vi "Measurement Logic.vi"() -> ()   [LabVIEW 2022 SP3, in "Single Tone - Digital Mic.lvlib"]
uses:
  Single Tone - Digital Mic.lvlib
  <vilib>/Plug-In SDKs/Measurements/Measure Call Context/Measure Call Context.lvclass
  Measurement Configuration.ctl
  shared/measurements/controls/lowpass filter.ctl
  shared/measurements/controls/weighting filter.ctl
  shared/measurements/controls/highpass filter.ctl
  shared/measurements/controls/measurement units.ctl
  Measurement Results.ctl
  <vilib>/addons/_NISVFA/_Generation/Signal Generation/SV Signal/sv_System Timing Model.ctl
  shared/Stop Variable Action.ctl
  <vilib>/PDM Acquisition Toolkit/host/Classes/Tasks/PDM Tasks/Controls/Acquisition Mode.ctl
  <vilib>/PDM Acquisition Toolkit/shared/controls/clock mode.ctl
  shared/measurements/controls/audio filter settings.ctl
  shared/measurements/controls/single tone microphone measurement settings.ctl
  shared/measurements/controls/units settings - mic.ctl
  <vilib>/DAQmx/read.llb/DAQmx Read (Analog Wfm 1Chan NSamp).vi
  <vilib>/DAQmx/write.llb/DAQmx Write (Analog Wfm 1Chan NSamp).vi
  <vilib>/addons/_NISVFA/_Generation/Signal Generation/SV Sinusoid/SV Sinusoid.lvclass
  C:/Program Files/National Instruments/LabVIEW 2022/vi.lib/addons/_NISVFA/_Generation/Signal Generation/SV Signal/SV Signal.lvclass
  <vilib>/addons/_NISVFA/_Generation/Signal Generation/SV Sinusoid/Configure Sine.vi
  <vilib>/DAQmx/create/channels.llb/DAQmx Create Channel (AO-Voltage-Basic).vi
  <vilib>/DAQmx/configure/timing.llb/DAQmx Timing (Sample Clock).vi
  <vilib>/DAQmx/configure/events/hardwareSignals.llb/DAQmx Export Signal (Most Signals).vi
  <vilib>/addons/_NISVFA/_Generation/Signal Generation/SV Signal/Write Sample Rate.vi
  <vilib>/addons/_NISVFA/_Generation/Signal Generation/SV Signal/Write System Timing Model.vi
  <vilib>/addons/_NISVFA/_Generation/Signal Generation/SV Signal/Write Ramp Parameters.vi
  <vilib>/DAQmx/create/channels.llb/DAQmx Create Channel (AI-Sound Pressure-Microphone).vi
  <vilib>/Waveform/WDTOps.llb/WDT Waveform Duration DBL.vi
  <vilib>/DAQmx/configure/trigger.llb/DAQmx Start Trigger (Digital Edge).vi
  <vilib>/DAQmx/miscellaneous.llb/DAQmx Fill In Error Info.vi
  <vilib>/Waveform/WDTOps.llb/WDT Get Waveform Subset DBL.vi
  <vilib>/addons/_NISVFA/_Generation/Signal Generation/SV Signal/SV Signal.lvclass
  <resource>/objmgr/daqmx.rc
  shared/combined digital api/Combo Digital Audio API.lvlib
  <vilib>/PDM Acquisition Toolkit/host/Classes/Tasks/PDM Tasks/PDM Task.lvclass
  <vilib>/PDM Acquisition Toolkit/shared/PDM Shared.lvlib
panel:
  out "calculated microphone sensitivity (dBFS)":dbl
  out "measurement results":T1={"channel name"="Empty", "frequency (Hz)"=0.0, "amplitude (Pa RMS)"=0.0, "amplitude (dBSPL)"=0.0, "microphone sensitivity (dBFS)"=0.0, "SNR"=0.0, "THD+N"=0.0, "THD"=0.0, "wfm - dt"=0.0, "wfm - data"=[0.0], "fft - f0"=0.0, "fft - df"=0.0, "fft - data"=[0.0], "ref mic wfm - dt"=0.0, "ref mic wfm - data"=[0.0]}
  in  "measurement configuration":T2={"digital channel list"="Lorem ipsum dolor sit", "input cfg file"="", "digital mic sensitivity (dBFS)"=1.2, "ref mic channel"="7821\\PCMo 0", "ref mic sensitivity (mV/Pa)"=32.0, "output channel"="7821\\PCMo 0", "signal frequency"=64.0, "output level (dBSPL)"=-32.0, "output voltage ratio"=-64.0, "lowpass filter"=enum."No filter", "weighting filter"=enum."A-weighting", "highpass filter"=enum."AC", "band start"=1.0, "band stop"=1.0, "min measurement cycles"=20, "min measurement time (s)"=0.1, "min settling cycles"=0, "min settling time (s)"=0.0, "SNR units"=enum."dB", "THD+N units"=enum."dB", "THD units"=enum."dB"} {"output voltage ratio" format="%#_g Pa/V"; "signal frequency" format="%#_13g"; "digital mic sensitivity (dBFS)" format="%#_13g"}
  out "measure call context out":refnum<class "Measure Call Context.lvclass">
  in  "measure call context in":refnum<class "Measure Call Context.lvclass">
  out "error out":errorcluster
  in  "error in":errorcluster
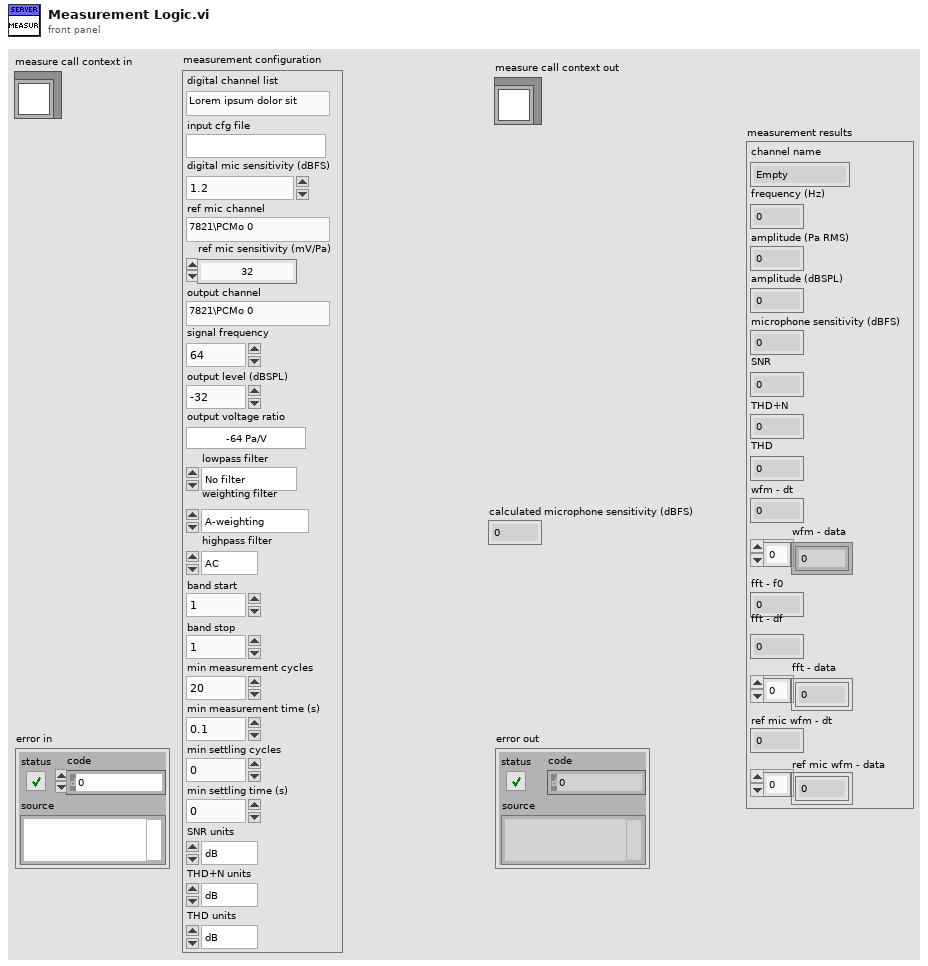
[diagram p1: front panel]
types:
  T1 = typedef "Single Tone - Digital Mic.lvlib/Measurement Results.ctl" = cluster{"channel name":string, "frequency (Hz)":dbl, "amplitude (Pa RMS)":dbl, "amplitude (dBSPL)":dbl, "microphone sensitivity (dBFS)":dbl, "SNR":dbl, "THD+N":dbl, "THD":dbl, "wfm - dt":dbl, "wfm - data":dbl[], "fft - f0":dbl, "fft - df":dbl, "fft - data":dbl[], "ref mic wfm - dt":dbl, "ref mic wfm - data":dbl[]}
  T2 = typedef "Single Tone - Digital Mic.lvlib/Measurement Configuration.ctl" = cluster{"digital channel list":string, "input cfg file":string, "digital mic sensitivity (dBFS)":dbl, "ref mic channel":string, "ref mic sensitivity (mV/Pa)":dbl, "output channel":string, "signal frequency":dbl, "output level (dBSPL)":dbl, "output voltage ratio":dbl, "lowpass filter":T3, "weighting filter":T4, "highpass filter":T5, "band start":dbl, "band stop":dbl, "min measurement cycles":u32, "min measurement time (s)":dbl, "min settling cycles":u32, "min settling time (s)":dbl, "SNR units":T6, "THD+N units":T6, "THD units":T6}
  T3 = typedef "lowpass filter.ctl" = enum32{"No filter", "AES17 20kHz", "AES17 40kHz"}
  T4 = typedef "weighting filter.ctl" = enum32{"Linear", "A-weighting", "B-weighting", "C-weighting"}
  T5 = typedef "highpass filter.ctl" = enum32{"DC", "AC"}
  T6 = typedef "measurement units.ctl" = enum32{"dB", "%", "x/y"}
  T7 = typedef "units settings - mic.ctl" = cluster{"SNR units":T6, "THD+N units":T6, "THD units":T6}
  T8 = typedef "single tone microphone measurement settings.ctl" = cluster{"Band start":dbl, "Band stop":dbl, "Frequency":dbl}
  T9 = typedef "audio filter settings.ctl" = cluster{"weighting filter":T4, "highpass filter":T5, "lowpass filter ":T3}
  T10 = typedef "PDM Shared.lvlib/clock mode.ctl" = enum16{"divided clock", "DDS"}
  T11 = typedef "PDM Acquisition Class Library.lvlib/PDM Task.lvclass/Acquisition Mode.ctl" = enum16{"Finite", "Continuous"}
  T12 = typedef "Stop Variable Action.ctl" = enum16{"Reset", "Check", "Stop"}
  T13 = typedef "SV Signal.lvclass/sv_System Timing Model.ctl" = i64
  T14 = cluster{"profile":enum16{"Linear", "Half cosine"}, "durations [s]":cluster{"ramp-up":dbl, "transition":dbl, "ramp-down":dbl}}
  T15 = typedef "Combo Digital Audio API.lvlib/task.ctl" = cluster{"task ref":u64, "audio type":T16, "sample rate":dbl}
  T16 = typedef "input type.ctl" = enum32{"Digital Serial", "PDM"}
  T17 = typedef "single tone microphone measurements.ctl" = cluster{"channel":string, "frequency (Hz)":dbl, "amplitude (Pa rms)":dbl, "amplitude (dBSPL)":dbl, "SNR":dbl, "THD+N":dbl, "THD":dbl, "phase (deg)":dbl}
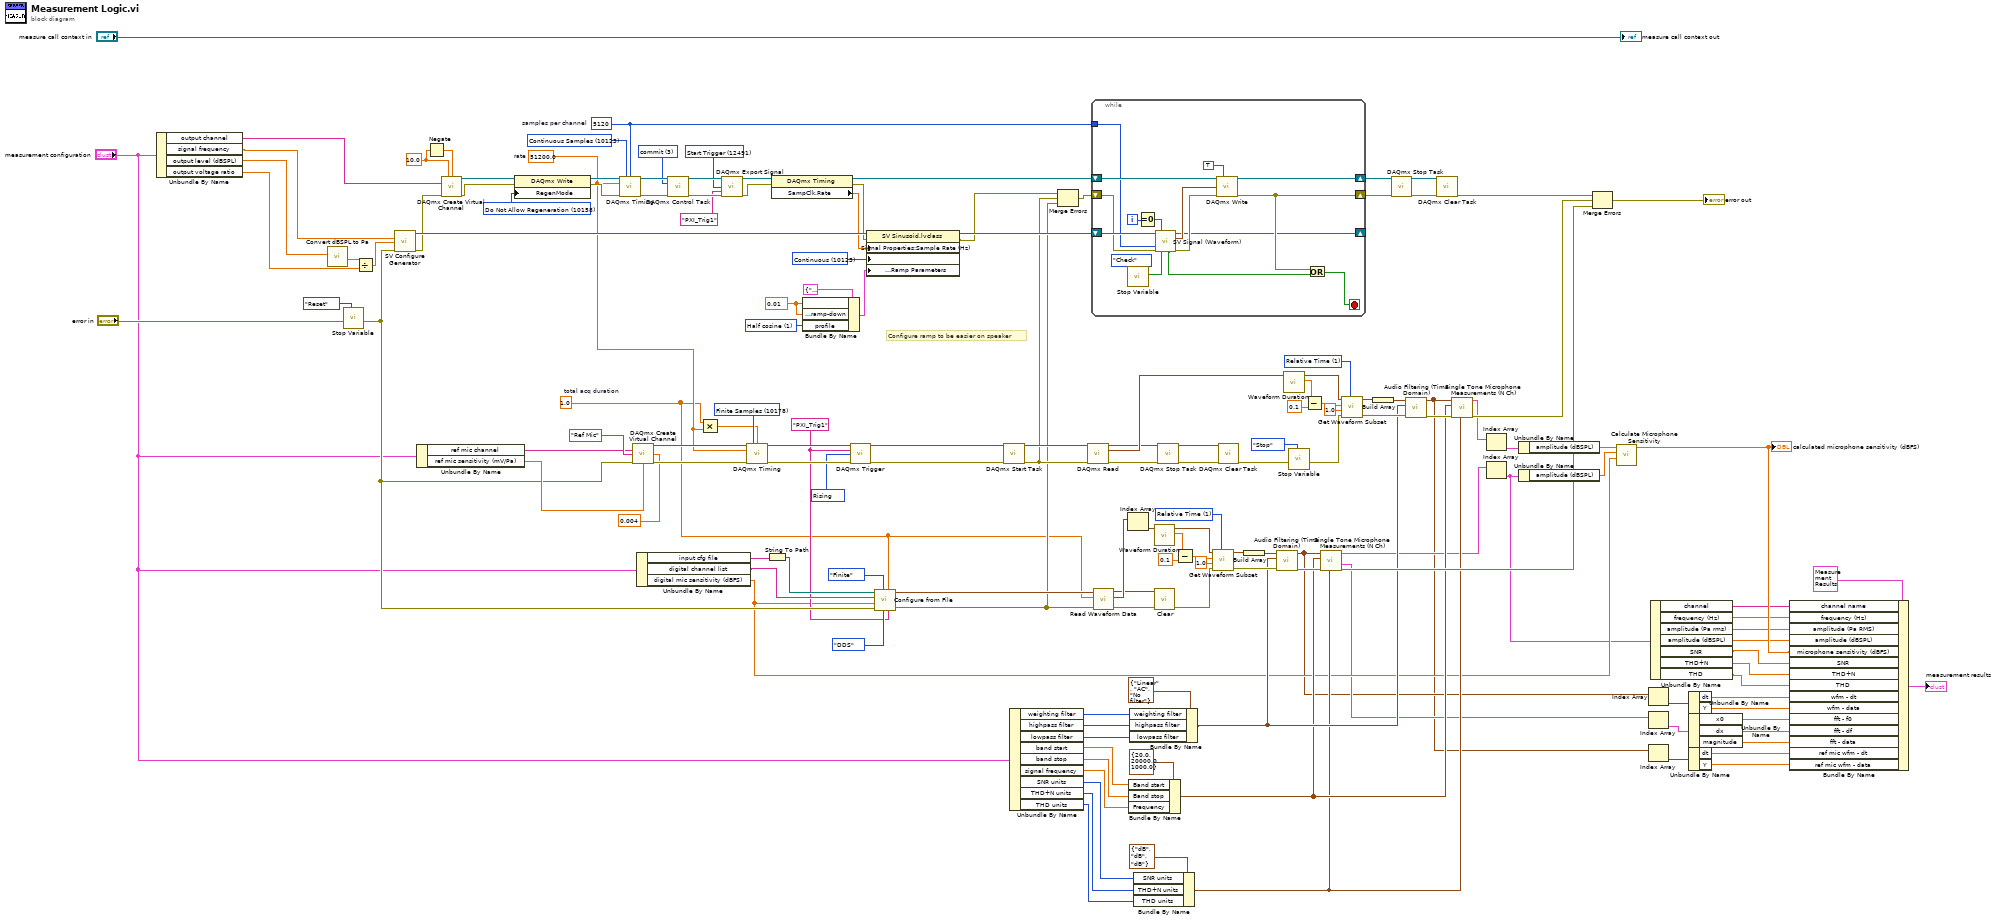
[diagram p0: block diagram]
diagram:
  w63 = u16 1 items=["Samples", "Relative Time"] ("start/duration format")
  w3 = 1.0  # total acq duration
  w92 = u16 1 items=["Samples", "Relative Time"] ("start/duration format")
  w104 = 10280 items=["Rising"=10280, "Falling"=10171] ("edge")
  w73 = "PXI_Trig1"
  w111 = 10178 items=["Finite Samples"=10178, "Continuous Samples"=10123] ("sample mode")
  w126 = 12491 items=["AI Convert Clock"=12484, "10MHz Reference Clock"=12536, "20MHz Timebase Clock"=12486, "Sample Clock"=12487, "Advance Trigger"=12488, "Reference Trigger"=12490, "Start Trigger"=12491, "Advance Complete Event"=12492, "AI Hold Complete Event"=12493, "Counter Output Event"=12494, "Change Detection Event"=12511, "Watchdog Timer Expired Event"=12512] ("signal")
  w131 = 3 items=["verify"=2, "reserve"=4, "commit"=3, "unreserve"=5, "abort"=6] ("action")
  w150 = 0.01 ("ramp duration")
  w148 = u16 1 items=["Linear", "Half cosine"] ("ramp profile")
  w142 = 10158 items=["Allow Regeneration"=10097, "Do Not Allow Regeneration"=10158] ("RegenMode")
  w145 = 10.0 ("maximum value")
  w112 = 5120  # samples per channel
  w146 = 10123 items=["Finite Samples"=10178, "Continuous Samples"=10123, "Hardware Timed Single Point"=12522] ("sample mode")
  w69 = 51200.0  # rate
  w147 = T13 10123 items=["Finite"=10178, "-"=-1, "Continuous"=10123, "-"=-2, "Settled"=110123, "Averaged"=210123, "Discrete Sweep"=310123, "Continuous Sweep"=410123] ("System Timing Model")
  # "Configure ramp to be easier on speaker"
  n1 = Unbundle By Name("measurement configuration") -> ("output channel"=w122:string, "signal frequency"=w121:dbl, "output level (dBSPL)"=w120:dbl, "output voltage ratio"=w119:dbl)
  n2 = call "Convert dBSPL to Pa.vi"("dB SPL"=w120) -> ("Pa pk"=w135:dbl)  [unwired: 9 in, 1 out]
  n3 = call "Stop Variable.vi"("action"=Stop_Variable_Action."Reset", "error in (no error)"="error in") -> ("error out"=w77:errorcluster)  [unwired: 8 in, 1 out]
  n4 = Divide(x=w135, y=w119) -> (x/y=w134:dbl)
  n5 = call-poly <vilib>:"SV Configure Generator.vi"("frequency (Hz)"=w121, "amplitude"=w134, "error in (no error)"=w77) -> ("signal configuration"=w152:refnum<class "SV Sinusoid.lvclass">, "error out"=w143:errorcluster)  [unwired: 11 in]
  n6 = Unbundle By Name("measurement configuration") -> ("ref mic channel"=w102:string, "ref mic sensitivity (mV/Pa)"=w101:dbl)
  n7 = Negate(x=w145) -> (-x=w144:dbl)
  n8 = call-poly <vilib>:"DAQmx Create Virtual Channel.vi"("maximum value"=w145, "minimum value"=w144, "physical channels"=w122, "error in"=w143) -> ("task out"=w141:refnum<k21>, "error out"=w139:errorcluster)  [unwired: 10 in]
  n9 = property class="DAQmx Write"(reference=w141, error in=w139, "RegenMode"=w142) -> (reference out=w140:refnum<k21>, error out=w138:errorcluster)
  n10 = call-poly <vilib>:"DAQmx Timing.vi"("task/channels in"=w140, "sample mode"=w146, "samples per channel"=w112, "rate"=w69, "error in"=w138) -> ("task out"=w133:refnum<k21>, "error out"=w132:errorcluster)  [unwired: 9 in]
  n11 = call-poly <vilib>:"DAQmx Create Virtual Channel.vi"("physical channels"=w102, "name to assign"="Ref Mic", "current excitation value"=0.004, "error in"=w77, "microphone sensitivity"=w101) -> ("task out"=w110:refnum<k21>, "error out"=w109:errorcluster)  [unwired: 9 in]
  n12 = Unbundle By Name("measurement configuration") -> ("input cfg file"=w79:string, "digital channel list"=w76:string, "digital mic sensitivity (dBFS)"=w29:dbl)
  n13 = call <vilib>:"DAQmx Control Task.vi"("task/channels in"=w133, "action"=w131, "error in"=w132) -> ("task out"=w130:refnum<k21>, "error out"=w129:errorcluster)  [unwired: 11 in]
  n14 = Multiply(x=w3, y=w69) -> (x*y=w70:dbl)
  n15 = call-poly <vilib>:"DAQmx Export Signal.vi"("task/channels in"=w130, "signal"=w126, "output terminal"="PXI_Trig1", "error in"=w129) -> ("task out"=w128:refnum<k21>, "error out"=w127:errorcluster)  [unwired: 10 in]
  n16 = call-poly <vilib>:"DAQmx Timing.vi"("task/channels in"=w110, "sample mode"=w111, "samples per channel"=w70, "rate"=w69, "error in"=w109) -> ("task out"=w108:refnum<k21>, "error out"=w106:errorcluster)  [unwired: 9 in]
  n17 = String To Path(string=w79) -> (path=w78:path)
  n18 = property class="DAQmx Timing"(reference=w128, error in=w127) -> (reference out=w114:refnum<k21>, error out=w136:errorcluster, "SampClk.Rate"=w137:dbl)
  n19 = Bundle By Name(cluster=T14 {"profile"=enum."Linear", "durations [s]"={"ramp-up"=0.0, "transition"=0.0, "ramp-down"=0.0}} ("Ramp Parameters:All Elements"), "durations [s].ramp-up"=w150, "durations [s].ramp-down"=w150, "profile"=w148) -> (w149:T14)
  n20 = call-poly <vilib>:"DAQmx Trigger.vi"("task/channels in"=w108, "source"=w73, "edge"=w104, "error in"=w106) -> ("task out"=w107:refnum<k21>, "error out"=w105:errorcluster)  [unwired: 10 in]
  n21 = property class="SV Sinusoid.lvclass"(reference=w152, error in=w136, "Signal Properties:Sample Rate (Hz)"=w137, "Signal Properties:System Timing Model"=w147, "Signal Properties:Ramps:Ramp Parameters"=w149) -> (reference out=w113:refnum<class "SV Sinusoid.lvclass">, error out=w98:errorcluster)
  n22 = call "Configure from File.vi"("digital trigger"=w73, "acq duration (s)"=w3, "clock mode"=clock_mode."DDS", "acquisition mode"=Acquisition_Mode."Finite", "error in (no error)"=w77, "microphone sensitivity (dBFS)"=w29, "channels"=w76, "file path"=w78) -> ("error out"=w71:errorcluster, "task"=w72:T15)  [unwired: 2 in]
  n23 = call <vilib>:"DAQmx Start Task.vi"("task/channels in"=w107, "error in"=w105) -> ("task out"=w90:refnum<k21>, "error out"=w89:errorcluster)  [unwired: 12 in]
  n24 = Unbundle By Name("measurement configuration") -> ("weighting filter"=w47:T4, "highpass filter"=w46:T5, "lowpass filter"=w45:T3, "band start"=w42:dbl, "band stop"=w41:dbl, "signal frequency"=w1:dbl, "SNR units"=w2:T6, "THD+N units"=w36:T6, "THD units"=w35:T6)
  n25 = Merge Errors(w98, w89, w71) -> (w99:errorcluster)
  n26 = call-poly <vilib>:"DAQmx Read.vi"("task/channels in"=w90, "error in"=w89) -> ("task out"=w84:refnum<k21>, "data"=w91:waveform(dbl), "error out"=w51:errorcluster)  [unwired: 11 in]
  n27 = while {
    tunnel: w112 -> [w167]
    shift-right: [w165] -> w118
    shift-left: w114 -> [w169]
    shift-right: [w166] -> w117
    shift-left: w99 -> [w161]
    shift-right: [w160] -> _
    shift-left: w113 -> [w168]
    i -> [w157]
    stop <- w159 stop-if-true
    n28 = call "Stop Variable.vi"("action"=Stop_Variable_Action."Check") -> ("stop"=w155:bool)  [unwired: 9 in, 1 out]
    n29 = Equal To 0?(x=w157) -> (x = 0?=w158:bool)
    n30 = call-dynamic "SV Signal (Waveform).vi"("signal configuration"=w168, "reset"=w158, "samples"=w167, "error in (no error)"=w161, "stop"=w155) -> ("signal configuration"=w160:refnum<class "SV Sinusoid.lvclass">, "output waveform"=w163:waveform(dbl), "done"=w156:bool, "error out"=w164:errorcluster)  [unwired: 5 in, 2 out]
    n31 = call-poly <vilib>:"DAQmx Write.vi"("task/channels in"=w169, "auto start"=TRUE, "data"=w163, "error in"=w164) -> ("task out"=w165:refnum<k21>, "error out"=w166:errorcluster)  [unwired: 9 in, 1 out]
    n32 = Or(x=w166, y=w156) -> (x .or. y?=w159:bool)
  }
  n33 = call "Read Waveform Data.vi"("error in (no error)"=w71, "acq duration (s)"=w3, "task"=w72) -> ("error out"=w55:errorcluster, "waveforms"=w60:waveform(dbl)[], "task"=w54:T15)  [unwired: 6 in]
  n34 = Index Array(array=w60) -> (element=w61:waveform(dbl))  [unwired: 1 in]
  n35 = Bundle By Name(cluster=T8 {"Band start"=20.0, "Band stop"=20000.0, "Frequency"=1000.0} ("measurement settings"), "Band start"=w42, "Band stop"=w41, "Frequency"=w1) -> (w39:T8)
  n36 = Bundle By Name(cluster=T9 {"weighting filter"=enum."Linear", "highpass filter"=enum."AC", "lowpass filter "=enum."No filter"} ("filter settings"), "weighting filter"=w47, "highpass filter"=w46, "lowpass filter"=w45) -> (w40:T9)
  n37 = Bundle By Name(cluster=T7 {"SNR units"=enum."dB", "THD+N units"=enum."dB", "THD units"=enum."dB"} ("units settings"), "SNR units"=w2, "THD+N units"=w36, "THD units"=w35) -> (w37:T7)
  n38 = call-poly <vilib>:"Waveform Duration.vi"("waveform in"=w61) -> ("duration"=w68:dbl, "waveform out"=w64:waveform(dbl))  [unwired: 8 in, 1 out]
  n39 = call "Clear.vi"("error in (no error)"=w55, "task"=w54) -> ("error out"=w53:errorcluster)  [unwired: 9 in]
  n40 = call <vilib>:"DAQmx Stop Task.vi"("task/channels in"=w84, "error in"=w51) -> ("task out"=w88:refnum<k21>, "error out"=w87:errorcluster)  [unwired: 12 in]
  n41 = Subtract(x=w68, y=0.1) -> (x-y=w65:dbl)
  n42 = call-poly <vilib>:"Get Waveform Subset.vi"("start/duration format"=w63, "error in (no error)"=w53, "duration"=1.0, "start samples/time"=w65, "waveform in"=w64) -> ("error out"=w57:errorcluster, "waveform out"=w62:waveform(dbl))  [unwired: 1 in, 2 out]
  n43 = call <vilib>:"DAQmx Clear Task.vi"("task in"=w88, "error in"=w87) -> ("error out"=w85:errorcluster)  [unwired: 13 in]
  n44 = Build Array(w62) -> (w24:waveform(dbl)[])
  n45 = call "Audio Filtering (Time Domain).vi"("waveforms"=w24, "filter settings"=w40, "error in"=w57) -> ("time domain"=w22:waveform(dbl)[], "error out"=w56:errorcluster)  [unwired: 6 in]
  n46 = call-poly <vilib>:"Waveform Duration.vi"("waveform in"=w91) -> ("duration"=w97:dbl, "waveform out"=w93:waveform(dbl))  [unwired: 8 in, 1 out]
  n47 = call "Stop Variable.vi"("action"=Stop_Variable_Action."Stop", "error in (no error)"=w85) -> ("error out"=w50:errorcluster)  [unwired: 8 in, 1 out]
  n48 = Subtract(x=w97, y=0.1) -> (x-y=w94:dbl)
  n49 = call "Single Tone Microphone Measurements (N Ch).vi"("units settings"=w37, "error in"=w56, "measurement settings"=w39, "waveforms"=w22) -> ("error out"=w52:errorcluster, "spectra"=w23:cluster{"x0":dbl, "dx":dbl, "magnitude":dbl[]}[], "measurements"=w31:T17[])  [unwired: 4 in, 1 out]
  n50 = call-poly <vilib>:"Get Waveform Subset.vi"("start/duration format"=w92, "error in (no error)"=w50, "duration"=1.0, "start samples/time"=w94, "waveform in"=w93) -> ("error out"=w59:errorcluster, "waveform out"=w80:waveform(dbl))  [unwired: 1 in, 2 out]
  n51 = Build Array(w80) -> (w81:waveform(dbl)[])
  n52 = call <vilib>:"DAQmx Stop Task.vi"("task/channels in"=w118, "error in"=w117) -> ("task out"=w116:refnum<k21>, "error out"=w115:errorcluster)  [unwired: 12 in]
  n53 = call "Audio Filtering (Time Domain).vi"("waveforms"=w81, "filter settings"=w40, "error in"=w59) -> ("time domain"=w15:waveform(dbl)[], "error out"=w58:errorcluster)  [unwired: 6 in]
  n54 = call <vilib>:"DAQmx Clear Task.vi"("task in"=w116, "error in"=w115) -> ("error out"=w83:errorcluster)  [unwired: 13 in]
  n55 = call "Single Tone Microphone Measurements (N Ch).vi"("units settings"=w37, "error in"=w58, "measurement settings"=w39, "waveforms"=w15) -> ("error out"=w49:errorcluster, "measurements"=w34:T17[])  [unwired: 4 in, 2 out]
  n56 = Index Array(array=w34) -> (element=w33:T17)  [unwired: 1 in]
  n57 = Index Array(array=w31) -> (element=w11:T17)  [unwired: 1 in]
  n58 = Unbundle By Name(w33) -> ("amplitude (dBSPL)"=w32:dbl)
  n59 = Unbundle By Name(w11) -> ("amplitude (dBSPL)"=w30:dbl)
  n60 = Merge Errors(w83, w49, w52) -> (→"error out":errorcluster)
  n61 = call "Calculate Microphone Sensitivity.vi"("microphone sensitivity (dBFS)"=w29, "measured sound level (dBSPL)"=w30, "reference sound level (dBSPL)"=w32) -> ("calculated microphone sensitivity (dBFS)"=w12:dbl)  [unwired: 8 in]
  "calculated microphone sensitivity (dBFS)" <- w12
  n62 = Index Array(array=w22) -> (element=w26:waveform(dbl))  [unwired: 1 in]
  n63 = Index Array(array=w23) -> (element=w25:cluster{"x0":dbl, "dx":dbl, "magnitude":dbl[]})  [unwired: 1 in]
  n64 = Index Array(array=w15) -> (element=w16:waveform(dbl))  [unwired: 1 in]
  n65 = Unbundle By Name(w11) -> ("channel"=w10:string, "frequency (Hz)"=w9:dbl, "amplitude (Pa rms)"=w8:dbl, "amplitude (dBSPL)"=w7:dbl, "SNR"=w6:dbl, "THD+N"=w5:dbl, "THD"=w4:dbl)
  n66 = Unbundle By Name(w26) -> ("dt"=w21:dbl, "Y"=w20:dbl[])
  n67 = Unbundle By Name(w25) -> ("x0"=w19:dbl, "dx"=w18:dbl, "magnitude"=w17:dbl[])
  n68 = Unbundle By Name(w16) -> ("dt"=w14:dbl, "Y"=w13:dbl[])
  n69 = Bundle By Name(cluster=T1 {"channel name"="Empty", "frequency (Hz)"=0.0, "amplitude (Pa RMS)"=0.0, "amplitude (dBSPL)"=0.0, "microphone sensitivity (dBFS)"=0.0, "SNR"=0.0, "THD+N"=0.0, "THD"=0.0, "wfm - dt"=0.0, "wfm - data"=[0.0], "fft - f0"=0.0, "fft - df"=0.0, "fft - data"=[0.0], "ref mic wfm - dt"=0.0, "ref mic wfm - data"=[0.0]} ("measurement results"), "channel name"=w10, "frequency (Hz)"=w9, "amplitude (Pa RMS)"=w8, "amplitude (dBSPL)"=w7, "microphone sensitivity (dBFS)"=w12, "SNR"=w6, "THD+N"=w5, "THD"=w4, "wfm - dt"=w21, "wfm - data"=w20, "fft - f0"=w19, "fft - df"=w18, "fft - data"=w17, "ref mic wfm - dt"=w14, "ref mic wfm - data"=w13) -> (→"measurement results":T1)
  "measure call context out" <- "measure call context in"
